vi "CSM - Start Watchdog to Ensure All Modules Exit.vi"(8 "error in (no error)":errorcluster) -> (0 "error out":errorcluster)   [LabVIEW 2017, in "CSM Watchdog.lvlib"]
doc: "Starts the CSM Watchdog thread to monitor whether the main program has exited. It is typically executed immediately after the main program starts.\n\n<b>Application Scenario</b>: Used to ensure that all asynchronously started CSM modules can exit normally after the main program exits.\n\n\n> [!NOTE] <b>CSM WatchDog Implementation Principle</b>\n>\n> When a LabVIEW VI exits, it automatically releases all handle resources such as queues and events. Therefore, you can create a WatchDog thread that monitors a queue resource created by the main program VI. When this queue resource is released after the main VI exits, the WatchDog thread is triggered to send `Macro: Exit` to any CSM modules that have not yet exited, ensuring they exit normally."
uses:
  CSM Watchdog.lvlib
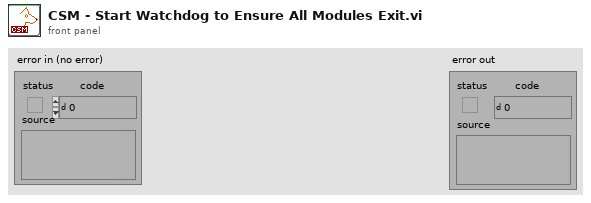
[diagram p1: front panel]
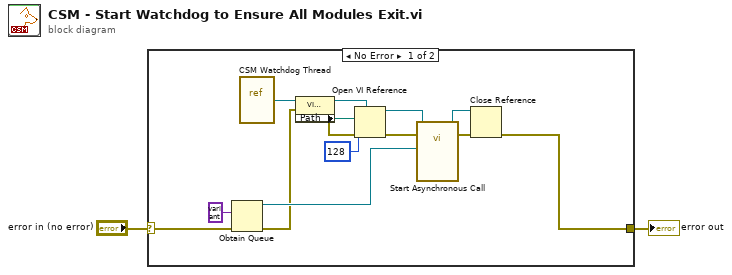
[diagram p0: block diagram]
diagram:
  n1 = case shown="No Error" "error in (no error)" {
    selector: "error in (no error)" -> [w4 w17]
    tunnel: [w7 w17] -> w1
    frame No Error {
      n2 = Obtain Queue(element data type=variant, error in (no error)=w4) -> (queue out=w5:refnum<queue>, error out=w3:errorcluster)  [unwired: 3 in, 1 out]
      n3 = vi-ref "CSM Watchdog Thread.vi"() -> (w10:refnum<vi>)
      n4 = property class="VI (strict)"(reference=w10, error in=w3) -> (reference out=w14:refnum<vi>, error out=w12:errorcluster, "Path"=w11:path)
      n5 = Open VI Reference(type specifier VI Refnum (for type only)=w14, vi path=w11, options=128, error in (no error)=w12) -> (vi reference=w9:refnum<vi>, error out=w15:errorcluster)  [unwired: 2 in]
      n6 = call-by-ref "Start Asynchronous Call"(reference=w9, error in=w15, "WatchdogQ"=w5) -> (reference out=w8:refnum<vi>, error out=w13:errorcluster)  [unwired: 11 in]
      n7 = Close Reference(reference=w8, error in (no error)=w13) -> (error out=w7:errorcluster)
    }
    frame Error {
    }
  }
  "error out" <- w1
